vi "Match Window to TabControl.vi"(9 "Tab Control":refnum<vi>, 10 "Pane":refnum<vi>, 11 "VI in":refnum<vi>) -> ()   [LabVIEW 2020, in "Data Viewer.lvlib" / "Data Viewer.lvclass"]
uses:
  Data Viewer.lvclass
  <vilib>/Utility/miscctls.llb/LVPositionTypeDef.ctl
  <vilib>/Utility/miscctls.llb/LVPointTypeDef.ctl
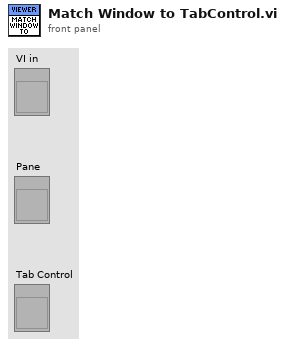
[diagram p1: front panel]
types:
  T1 = typedef "LVPointTypeDef.ctl" = cluster{"Horizontal":i16, "Vertical":i16}
  T2 = typedef "LVPositionTypeDef.ctl" = cluster{"Left":i32, "Top":i32}
  T3 = typedef "LVBoundsTypeDef.ctl" = cluster{"Width":u32, "Height":u32}
  T4 = typedef "LVRectTypeDef.ctl" = cluster{"Left":i16, "Top":i16, "Right":i16, "Bottom":i16}
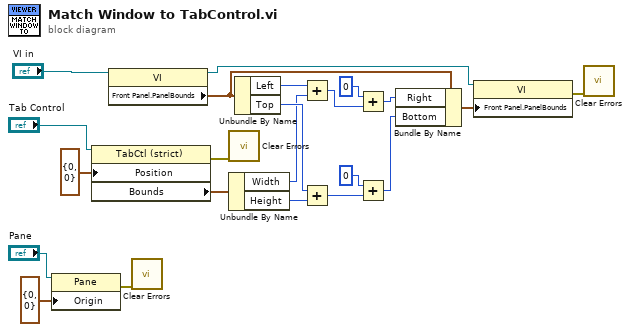
[diagram p0: block diagram]
diagram:
  n1 = property class="Pane"(reference="Pane", "Origin"=T1 {"Horizontal"=0, "Vertical"=0}) -> (error out=w20:errorcluster)  [unwired: 1 in, 1 out]
  n2 = property class="TabCtl (strict)"(reference="Tab Control", "Position"=T2 {"Left"=0, "Top"=0} ("位置")) -> (error out=w22:errorcluster, "Bounds"=w9:T3)  [unwired: 1 in, 1 out]
  n3 = property class="VI"(reference="VI in") -> (reference out=w6:refnum<vi>, "Front Panel.PanelBounds"=w7:T4)  [unwired: 1 in, 1 out]
  n4 = call <vilib>:"Clear Errors.vi"("error in (no error)"=w20) -> ()  [unwired: 5 in, 2 out]
  n5 = call <vilib>:"Clear Errors.vi"("error in (no error)"=w22) -> ()  [unwired: 5 in, 2 out]
  n6 = Unbundle By Name(w9) -> ("Width"=w10:u32, "Height"=w13:u32)
  n7 = Unbundle By Name(w7) -> ("Left"=w8:i16, "Top"=w12:i16)
  n8 = Add(x=w8, y=w10) -> (x+y=w11:u32)
  n9 = Add(x=w12, y=w13) -> (x+y=w14:u32)
  n10 = Add(x=u32 0, y=w11) -> (x+y=w4:u32)
  n11 = Add(x=u32 0, y=w14) -> (x+y=w2:u32)
  n12 = Bundle By Name(cluster=w7, "Right"=w4, "Bottom"=w2) -> (w15:T4)
  n13 = property class="VI"(reference=w6, "Front Panel.PanelBounds"=w15) -> (error out=w21:errorcluster)  [unwired: 1 in, 1 out]
  n14 = call <vilib>:"Clear Errors.vi"("error in (no error)"=w21) -> ()  [unwired: 5 in, 2 out]
